vi "RemoteVI Pack Point lParam.vi"(0 "x":i32, 5 "y":i32) -> (4 "lParam":i64)   [LabVIEW 2020, in "RemoteVI.lvlib"]
doc: "Packs a point into a mouse message lParam as Windows does (MAKELPARAM): (y AND 0xFFFF) * 65536 + (x AND 0xFFFF). Negative coordinates keep their low 16 bits. Pure."
uses:
  RemoteVI.lvlib
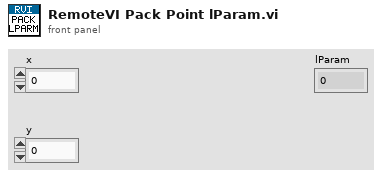
[diagram p1: front panel]
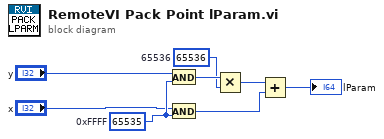
[diagram p0: block diagram]
diagram:
  w4 = i64 65536  # 65536
  w3 = 65535  # 0xFFFF
  n1 = And(x="y", y=w3) -> (x .and. y?=w6:i32)
  n2 = And(x="x", y=w3) -> (x .and. y?=w5:i32)
  n3 = Multiply(x=w6, y=w4) -> (x*y=w7:i64)
  n4 = Add(x=w7, y=w5) -> (x+y=→"lParam":i64)
